vi "DSS-test-roundtrip.vi"(8 "error in":errorcluster) -> (0 "error out":errorcluster)   [LabVIEW 2020, in "DSS-Tests.lvlib"]
doc: "Caraya test of RFH-save-common_format: reads ref_22p5c_water-mid.s2p, saves it to a unique file in the temporary directory, reads it back, deletes the file and checks every array is identical to the first read."
uses:
  DSS-Tests.lvlib
  <vilib>/addons/_JKI Toolkits/Caraya/classes/Test/Test.lvclass
  Reflector/RFH-Reflection_File_Handler.lvlib
  <vilib>/addons/_JKI Toolkits/Caraya/classes/Assert/Assert.lvclass
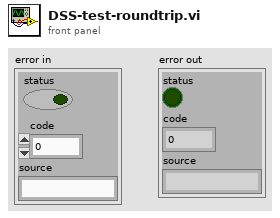
[diagram p1: front panel]
types:
  T1 = typedef "RFH-Reflection_File_Handler.lvlib/RFH-common_data_format.ctl" = cluster{"Frequency":dbl[], "Reflection'":dbl[], "Reflection''":dbl[], "Permativity'":dbl[], "Permativity''":dbl[], "Conductivity":dbl[], "Loss Tangent":dbl[], "Resistance":dbl[], "Reactance":dbl[]}
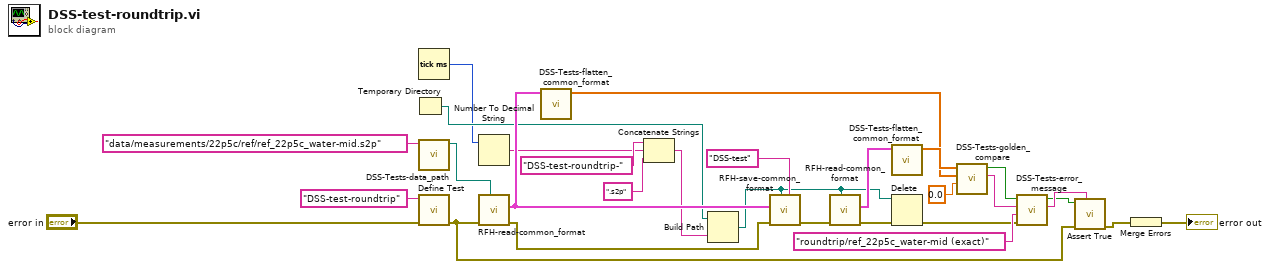
[diagram p0: block diagram]
diagram:
  n1 = Temporary Directory() -> (w9:path)
  n2 = Tick Count (ms)() -> (millisecond timer value=w4:u32)
  n3 = call "DSS-Tests-data_path.vi"("relative path"="data/measurements/22p5c/ref/ref_22p5c_water-mid.s2p") -> ("path"=w12:path)  [unwired: 10 in]
  n4 = call <vilib>:"Define Test.vi"("error in (no error)"="error in", "Label (VI Title)"="DSS-test-roundtrip") -> ("error out"=w3:errorcluster)  [unwired: 8 in, 1 out]
  n5 = Number To Decimal String(number=w4) -> (decimal integer string=w5:string)  [unwired: 1 in]
  n6 = call "RFH-read-common_format.vi"("file path (dialog if empty)"=w12, "error in"=w3) -> ("error out"=w13:errorcluster, "Common Format"=w14:T1)  [unwired: 8 in]
  n7 = call "DSS-Tests-flatten_common_format.vi"("Common Format"=w14) -> ("flat"=w20:dbl[])  [unwired: 10 in]
  n8 = Concatenate Strings("DSS-test-roundtrip-" ("prefix"), w5, ".s2p" ("extension")) -> (w8:string)
  n9 = Build Path(base path=w9, name or relative path=w8) -> (appended path=w10:path)
  n10 = call "RFH-save-common_format.vi"("source"="DSS-test", "file path (use dialog)"=w10, "error in (no error)"=w13, "Common Format"=w14) -> ("error out"=w16:errorcluster)  [unwired: 7 in]
  n11 = call "RFH-read-common_format.vi"("file path (dialog if empty)"=w10, "error in"=w16) -> ("error out"=w17:errorcluster, "Common Format"=w18:T1)  [unwired: 8 in]
  n12 = call "DSS-Tests-flatten_common_format.vi"("Common Format"=w18) -> ("flat"=w21:dbl[])  [unwired: 10 in]
  n13 = Delete(path (use dialog)=w10, error in=w17) -> (error out=w19:errorcluster)  [unwired: 3 in, 2 out]
  n14 = call "DSS-Tests-golden_compare.vi"("rel tol"=0.0, "golden"=w20, "actual"=w21) -> ("message"=w24:string, "pass"=w23:bool)  [unwired: 6 in, 1 out]
  n15 = call "DSS-Tests-error_message.vi"("error in"=w19, "prefix"="roundtrip/ref_22p5c_water-mid (exact)", "message in"=w24, "pass in"=w23) -> ("message"=w27:string, "pass"=w26:bool)  [unwired: 5 in, 1 out]
  n16 = call <vilib>:"Assert True.vi"("Label"=w27, "error in (no error)"=w3, "True?"=w26) -> ("error out"=w28:errorcluster)  [unwired: 7 in, 1 out]
  n17 = Merge Errors(w28) -> (→"error out":errorcluster)
